vi "DeepU Front Panel.vi"() -> ()   [LabVIEW 2019, in "Results.lvlib" / "DeepU Results.lvclass"]
uses:
  DeepU Results.lvclass
  DeepU Results.lvclass/DeepU Results.ctl
  Test Stands/DeepU/DeepU Test Stand.lvclass
panel:
  out "AC":waveform(dbl)(graph) caption="Acceleration"
  out "Velocity":dbl(knob) caption="Velocity RMS, mm/s" scale=0.0..8.0
  in  "Vel":bool
  in  "AC":bool
  in  "Stable Cond":bool
  out "Inlet Pressure 2":dbl(knob) caption="Bed Pressure, kPa (g)" scale=0.0..2.0
  out "PD23 3m":dbl caption="PD 03m" format="%10.0f"
  out "PD23 1m":dbl caption="PD 01m" format="%10.0f"
  out "PD23 2m":dbl caption="PD 02m" format="%10.0f"
  out "PDX 3m":dbl format="%#10.0f"
  out "dp J 3m":dbl format="%10.0f"
  out "PDX 2m":dbl format="%#10.0f"
  out "dp J 2m":dbl format="%10.0f"
  out "PDX 1m":dbl format="%#10.0f"
  out "dp J1m":dbl format="%10.0f"
  out "TC Unit 2":string
  in  "Std Dev":bool
  out "Numeric":dbl=1.0
  in  "x std_dev":dbl=3.0 min=2.0 max=3.0 step=1.0 format="%#.0f"
  out "PDX 3 std":dbl format="%#10.0f"
  out "PDX 2 std":dbl format="%#10.0f"
  out "PDX 1 std":dbl format="%#10.0f"
  out "PDX 0 std":dbl format="%#10.0f"
  out "PD23 4 std":dbl caption="PD 4 std" format="%10.0f"
  out "PD23 1 std":dbl caption="PD 1 std" format="%10.0f"
  out "PD23 2 std":dbl caption="PD 2 std" format="%10.0f"
  out "PD23 3 std":dbl caption="PD 3 std" format="%10.0f"
  out "PD23 0 std":dbl caption="PD 0 std" format="%10.0f"
  out "J 3 std":dbl format="%10.0f"
  out "J 1 std":dbl format="%10.0f"
  out "J 2 std":dbl format="%10.0f"
  out "Fan Temp":dbl format="%#.1f"
  out "Fan Temperature":dbl(slide) scale=0.0..200.0
  out "Inv Temp":u16 caption="Inv Temp, C"
  out "Fan rpm":u16
  out "Fan I":dbl caption="Fan I, A" format="%.1f"
  out "Fan Const":bool=TRUE
  out "In range?":bool
  out "Inlet Pressure":dbl(knob) caption="Bed Pressure, kPa (g)" scale=0.0..20.0
  out "TC Unit":string
  out "paa 2":dbl caption="p bed" format="%10.0f"
  out "paa 0":dbl caption="pb" format="%10.0f"
  out "dp J 3":dbl format="%10.0f"
  out "dp J 1":dbl format="%10.0f"
  out "dp J 2":dbl format="%10.0f"
  out "PDX 2":dbl format="%#10.0f"
  out "PDX 0":dbl caption="PDX in" format="%#10.0f"
  out "PDX 1":dbl format="%#10.0f"
  out "PDX 3":dbl format="%#10.0f"
  out "Gas Humidity":dbl caption="%RH" format="%#.1f"
  out "T2":dbl format="%#5.1f"
  out "T1":dbl format="%#5.1f"
  out "Adjusted":bool
  in  "Gas Flow SP":sgl caption="Gas Flow" min=0 max=372 step=1
  in  "auto Flow":bool
  in  "Fan Out Ctrl":dbl caption="Fan Output (2 - 200 Hz)" min=0.0 max=200.0 step=1.0 format="%6.2f"
  in  "Gas Speed SP":sgl caption="Gas Speed" min=0 max=300 step=1
  out "Fan Output":dbl(slide) scale=0.0..100.0
  in  "auto":bool
  out "Gas Flow":sgl caption="Gas Flow, l/s" format="%.1f"
  out "Gas Speed":sgl caption="Gas speed" format="%10.2f"
  out "PD23 3":dbl caption="PD 03" format="%10.0f"
  out "PD23 1":dbl caption="PD 01" format="%10.0f"
  out "PD23 0":dbl caption="PD in" format="%10.0f"
  out "PD23 2":dbl caption="PD 02" format="%10.0f"
  out "PD23 4":dbl caption="PD out" format="%10.0f"
  # "Pressure in Pa"
  # "mean"
  # "dp/m"
  # "Automatic"
  # "Manual"
  # "mean"
  # "std_dev"
  # "dp/m"
  # "%"
  # "C"
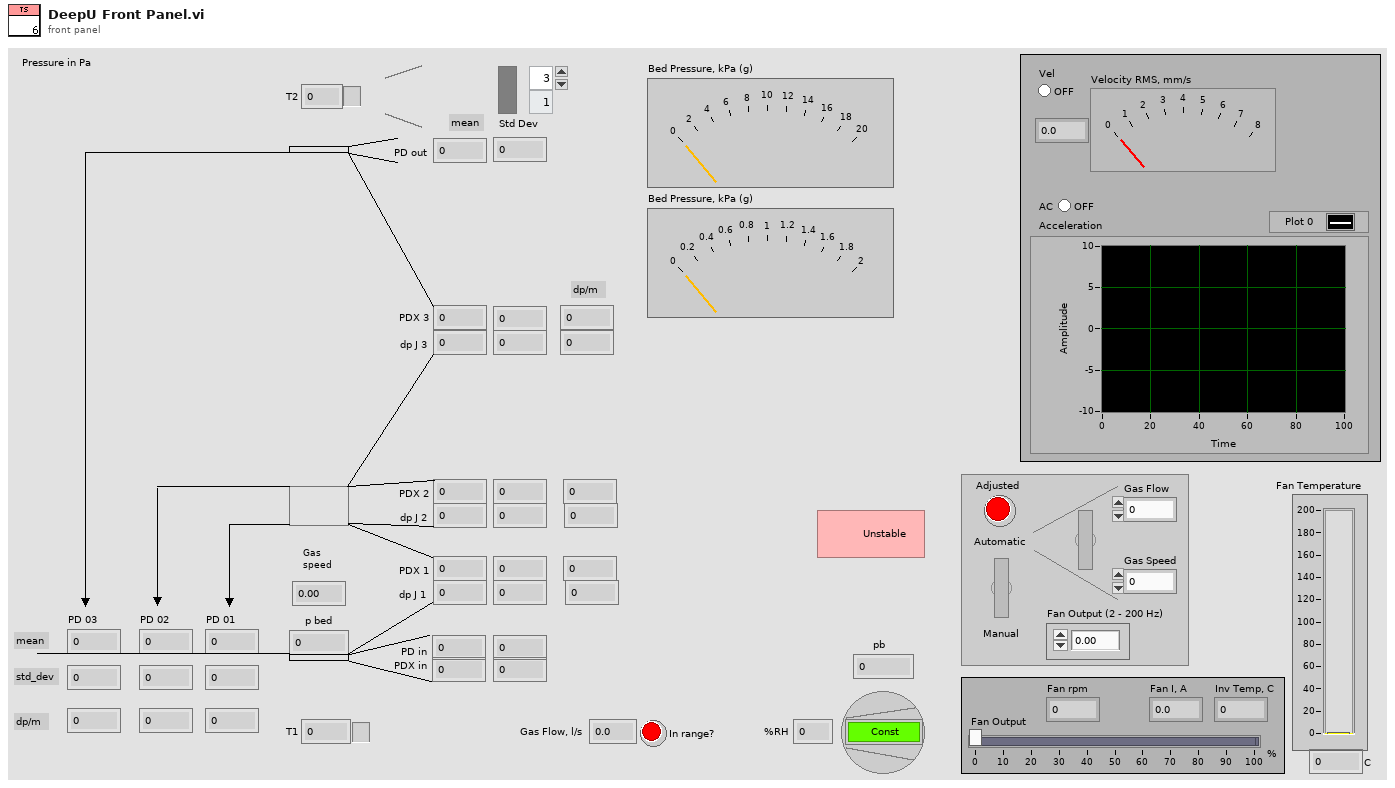
[diagram p1: front panel]
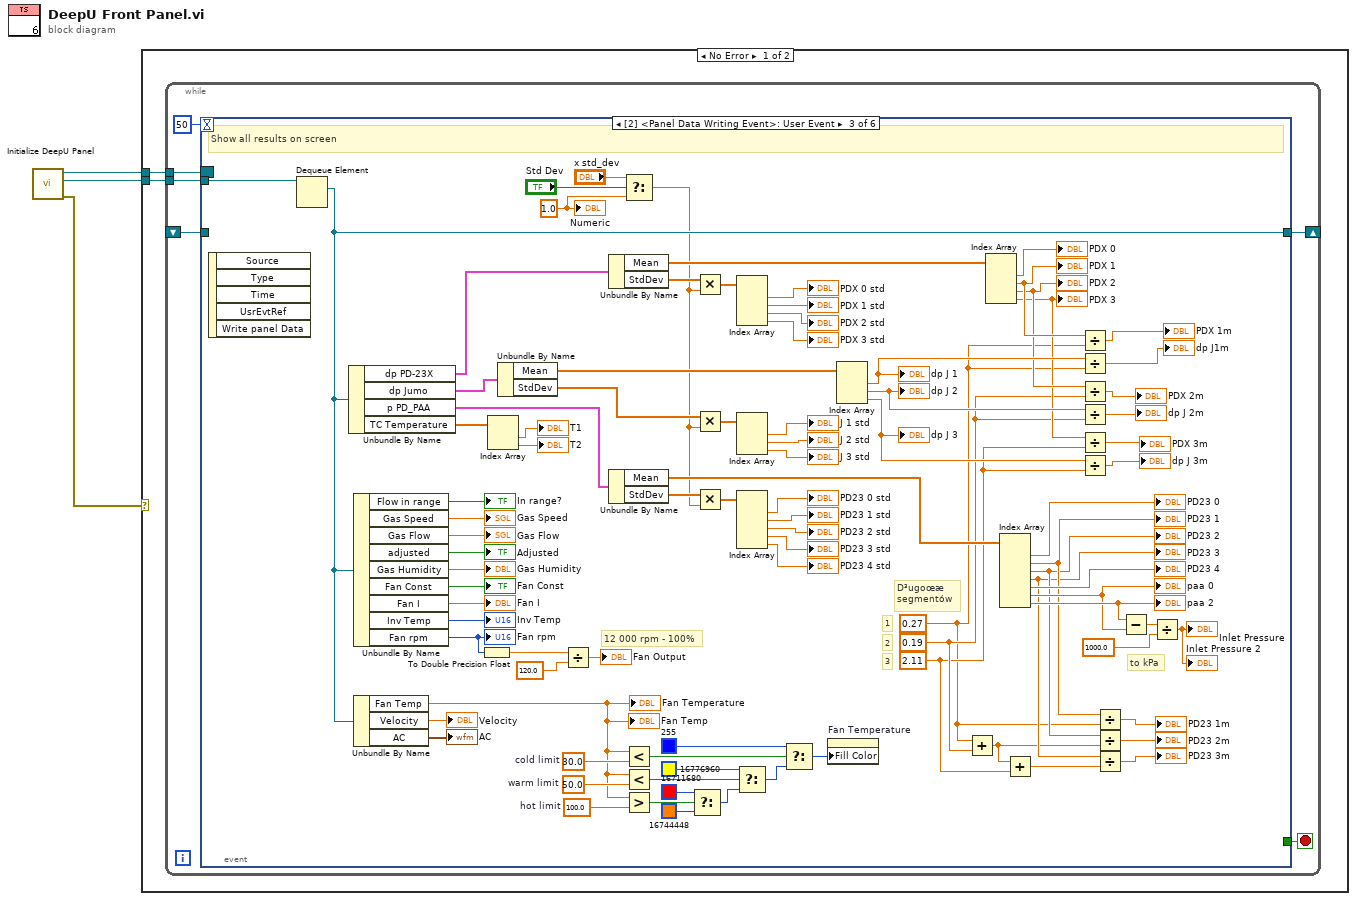
[diagram p0: block diagram]
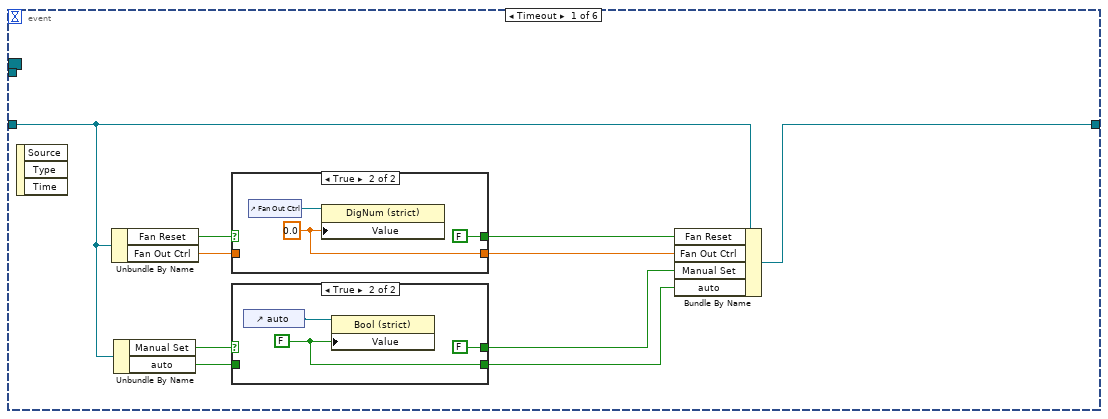
[diagram p2: hidden frame]
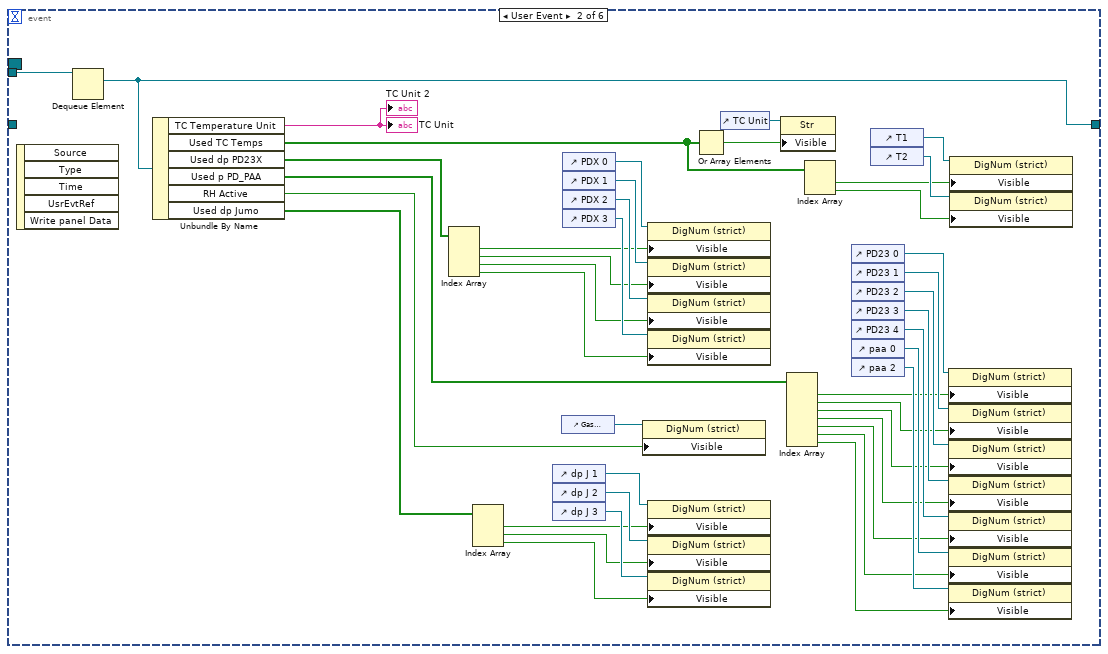
[diagram p5: hidden frame]
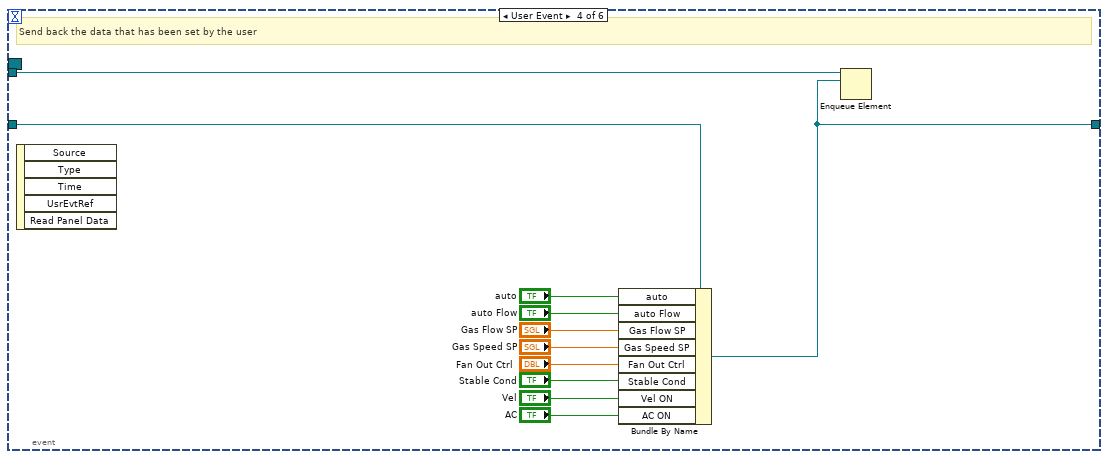
[diagram p6: hidden frame]
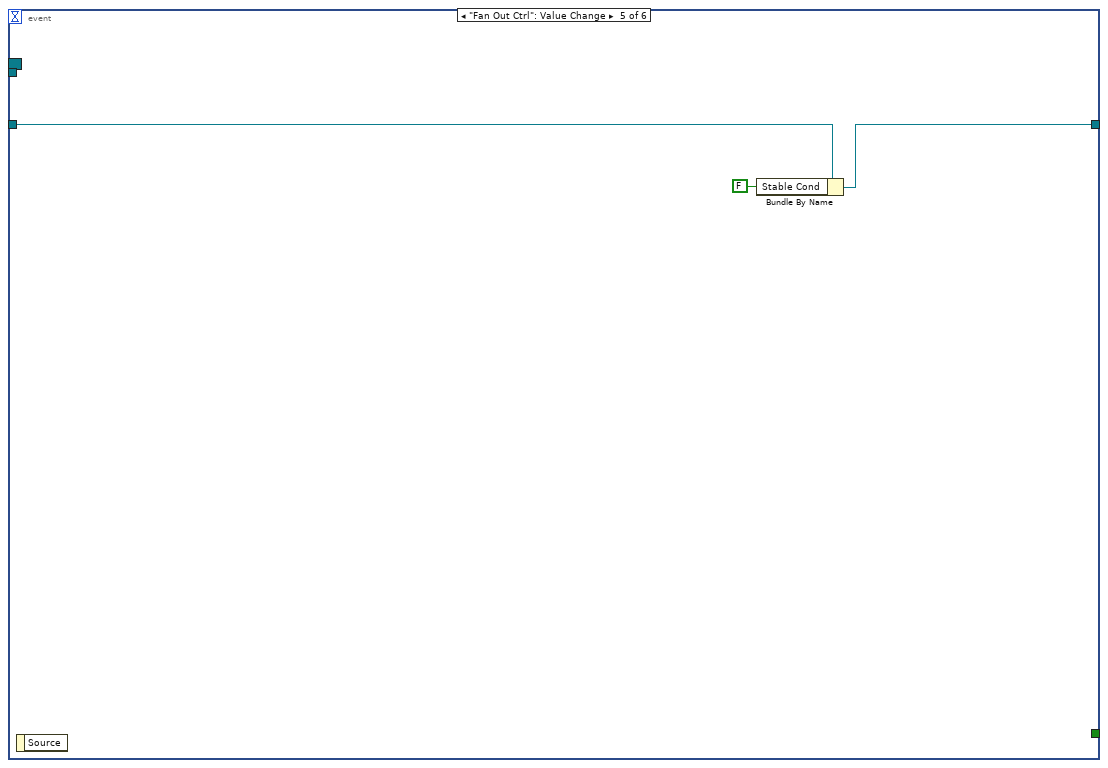
[diagram p7: hidden frame]
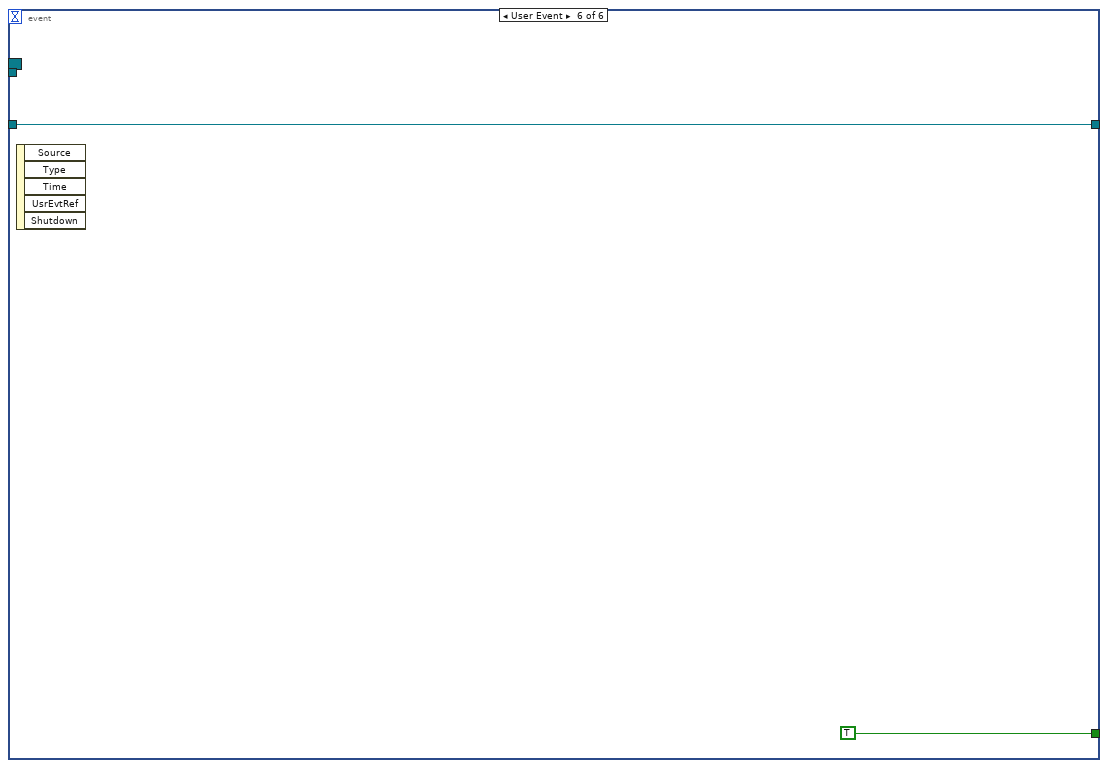
[diagram p8: hidden frame]
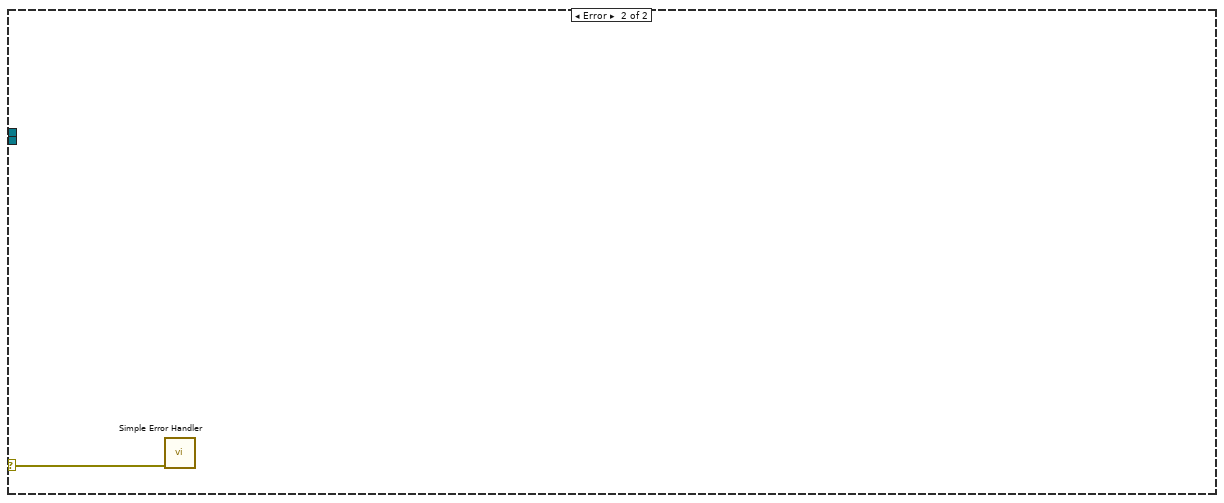
[diagram p9: hidden frame]
diagram:
  n1 = call "Initialize DeepU Panel.vi"() -> ("error out"=w3:errorcluster, "DeepU Results queue out"=w1:refnum<queue>, "Event Registration Refnum"=w2:refnum<event-registration>)  [unwired: 9 in]
  n2 = case shown="No Error" w3 {
    selector: w3 -> [_ w183]
    tunnel: w2 -> [w5 _]
    tunnel: w1 -> [w4 _]
    frame No Error {
      n3 = while {
        tunnel: w5 -> [w10]
        tunnel: w4 -> [w9]
        shift-right: [w7] -> _
        shift-left: _ -> [w6]
        stop <- w11 stop-if-true
        n4 = event shown="[2] <Panel Data Writing Event>: User Event" {
          selector: w10 -> [_ _ _ _ _ _]
          dyn-events: _ -> [_ _ _ _ _ _]
          timeout: 50 -> [_ _ _ _ _ _]
          tunnel: [_ _ _ _ _ TRUE] -> w11
          tunnel: w9 -> [_ w74 w166 w177 _ _]
          tunnel: [w21 w73 w148 w175 w179 w181] -> w7
          tunnel: w6 -> [w16 _ _ w176 w180 w181]
          event Timeout {
            n5 = event-data() -> ()  [unwired: 1 in, 3 out]
            n6 = Unbundle By Name(w16) -> ("Fan Reset"=w20:bool, "Fan Out Ctrl"=w19:dbl)
            n7 = Unbundle By Name(w16) -> ("Manual Set"=w15:bool, "auto"=w14:bool)
            n8 = case shown="True" w20 {
              selector: w20 -> [w27 _]
              tunnel: w19 -> [w28 _]
              tunnel: [w28 w29] -> w17
              tunnel: [w27 FALSE] -> w18
              frame False {
              }
              frame True {
                w29 = 0.0 ("t")
                n9 = control-ref of="Fan Out Ctrl"() -> (w31:refnum<vi>)
                n10 = property class="DigNum (strict)"(reference=w31, "Value"=w29) -> ()  [unwired: 1 in, 2 out]
              }
            }
            n11 = case shown="True" w15 {
              selector: w15 -> [w22 _]
              tunnel: w14 -> [w23 _]
              tunnel: [w23 w24] -> w12
              tunnel: [w22 FALSE] -> w13
              frame False {
              }
              frame True {
                w24 = FALSE
                n12 = control-ref of="auto"() -> (w25:refnum<vi>)
                n13 = property class="Bool (strict)"(reference=w25, "Value"=w24) -> ()  [unwired: 1 in, 2 out]
              }
            }
            n14 = Bundle By Name(cluster=w16, "Fan Reset"=w18, "Fan Out Ctrl"=w17, "Manual Set"=w13, "auto"=w12) -> (w21:refnum<class "DeepU Results.lvclass">)
          }
          event User Event {
            n15 = event-data() -> ()  [unwired: 1 in, 5 out]
            n16 = Dequeue Element(queue=w74) -> (element=w73:refnum<class "DeepU Results.lvclass">)  [unwired: 2 in, 3 out]
            n17 = Unbundle By Name(w73) -> ("TC Temperature Unit"=→"TC Unit" →"TC Unit 2":string, "Used TC Temps"=w69:bool[], "Used dp PD23X"=w64:bool[], "Used p PD_PAA"=w52:bool[], "RH Active"=w41:bool, "Used dp Jumo"=w37:bool[])
            n18 = Index Array(array=w64) -> (element #1=w63:bool, element #2=w62:bool, element #3=w61:bool, element #4=w60:bool)  [unwired: 4 in]
            n19 = Index Array(array=w37) -> (element #1=w36:bool, element #2=w35:bool, element #3=w34:bool)  [unwired: 3 in]
            n20 = control-ref of="dp J 1"() -> (w40:refnum<vi>)
            n21 = control-ref of="dp J 2"() -> (w39:refnum<vi>)
            n22 = control-ref of="dp J 3"() -> (w38:refnum<vi>)
            n23 = control-ref of="Gas Humidity"() -> (w44:refnum<vi>)
            n24 = control-ref of="PDX 0"() -> (w68:refnum<vi>)
            n25 = control-ref of="PDX 1"() -> (w67:refnum<vi>)
            n26 = control-ref of="PDX 2"() -> (w66:refnum<vi>)
            n27 = control-ref of="PDX 3"() -> (w65:refnum<vi>)
            n28 = property class="DigNum (strict)"(reference=w44, "Visible"=w41) -> ()  [unwired: 1 in, 2 out]
            n29 = property class="DigNum (strict)"(reference=w68, "Visible"=w63) -> ()  [unwired: 1 in, 2 out]
            n30 = property class="DigNum (strict)"(reference=w67, "Visible"=w62) -> ()  [unwired: 1 in, 2 out]
            n31 = property class="DigNum (strict)"(reference=w66, "Visible"=w61) -> ()  [unwired: 1 in, 2 out]
            n32 = property class="DigNum (strict)"(reference=w65, "Visible"=w60) -> ()  [unwired: 1 in, 2 out]
            n33 = property class="DigNum (strict)"(reference=w40, "Visible"=w36) -> ()  [unwired: 1 in, 2 out]
            n34 = property class="DigNum (strict)"(reference=w39, "Visible"=w35) -> ()  [unwired: 1 in, 2 out]
            n35 = property class="DigNum (strict)"(reference=w38, "Visible"=w34) -> ()  [unwired: 1 in, 2 out]
            n36 = Or Array Elements(Boolean array=w69) -> (logical OR=w43:bool)
            n37 = control-ref of="TC Unit"() -> (w72:refnum<vi>)
            n38 = property class="Str"(reference=w72, "Visible"=w43) -> ()  [unwired: 1 in, 2 out]
            n39 = Index Array(array=w52) -> (element #1=w51:bool, element #2=w45:bool, element #3=w46:bool, element #4=w47:bool, element #5=w48:bool, element #6=w49:bool, element #7=w50:bool)  [unwired: 7 in]
            n40 = Index Array(array=w69) -> (element #1=w42:bool, element #2=w33:bool)  [unwired: 2 in]
            n41 = control-ref of="PD23 0"() -> (w59:refnum<vi>)
            n42 = control-ref of="PD23 1"() -> (w58:refnum<vi>)
            n43 = control-ref of="PD23 2"() -> (w57:refnum<vi>)
            n44 = control-ref of="PD23 3"() -> (w56:refnum<vi>)
            n45 = control-ref of="PD23 4"() -> (w55:refnum<vi>)
            n46 = control-ref of="paa 0"() -> (w54:refnum<vi>)
            n47 = control-ref of="paa 2"() -> (w53:refnum<vi>)
            n48 = control-ref of="T1"() -> (w70:refnum<vi>)
            n49 = control-ref of="T2"() -> (w71:refnum<vi>)
            n50 = property class="DigNum (strict)"(reference=w59, "Visible"=w51) -> ()  [unwired: 1 in, 2 out]
            n51 = property class="DigNum (strict)"(reference=w58, "Visible"=w45) -> ()  [unwired: 1 in, 2 out]
            n52 = property class="DigNum (strict)"(reference=w57, "Visible"=w46) -> ()  [unwired: 1 in, 2 out]
            n53 = property class="DigNum (strict)"(reference=w56, "Visible"=w47) -> ()  [unwired: 1 in, 2 out]
            n54 = property class="DigNum (strict)"(reference=w55, "Visible"=w48) -> ()  [unwired: 1 in, 2 out]
            n55 = property class="DigNum (strict)"(reference=w54, "Visible"=w49) -> ()  [unwired: 1 in, 2 out]
            n56 = property class="DigNum (strict)"(reference=w53, "Visible"=w50) -> ()  [unwired: 1 in, 2 out]
            n57 = property class="DigNum (strict)"(reference=w70, "Visible"=w42) -> ()  [unwired: 1 in, 2 out]
            n58 = property class="DigNum (strict)"(reference=w71, "Visible"=w33) -> ()  [unwired: 1 in, 2 out]
          }
          event User Event {
            w80 = 2.11 ("y")
            w82 = 0.19 ("y")
            w78 = 0.27 ("y")
            w103 = 1.0 ("Numeric")
            w146 = 100.0  # hot limit
            w150 = 50.0  # warm limit
            w152 = 30.0  # cold limit
            # "3"
            # "2"
            # "1"
            # "D³ugoœæ\nsegmentów"
            # "to kPa"
            # "12 000 rpm - 100%"
            # "Show all results on screen"
            n59 = event-data() -> ()  [unwired: 1 in, 5 out]
            n60 = Dequeue Element(queue=w166) -> (element=w148:refnum<class "DeepU Results.lvclass">)  [unwired: 2 in, 3 out]
            n61 = Unbundle By Name(w148) -> ("dp PD-23X"=w162:cluster{"Mean":dbl[], "StdDev":dbl[]}, "dp Jumo"=w135:cluster{"Mean":dbl[], "StdDev":dbl[]}, "p PD_PAA"=w112:cluster{"Mean":dbl[], "StdDev":dbl[]}, "TC Temperature"=w111:dbl[])
            n62 = Unbundle By Name(w148) -> ("Flow in range"=→"In range?":bool, "Gas Speed"=→"Gas Speed":sgl, "Gas Flow"=→"Gas Flow":sgl, "adjusted"=→"Adjusted":bool, "Gas Humidity"=→"Gas Humidity":dbl, "Fan Const"=→"Fan Const":bool, "Fan I"=→"Fan I":dbl, "Inv Temp"=→"Inv Temp":u16, "Fan rpm"=w154:u16)
            "Fan rpm" <- w154
            n63 = Unbundle By Name(w148) -> ("Fan Temp"=w138:dbl, "Velocity"=→"Velocity":dbl, "AC"=→"AC":waveform(dbl))
            "Fan Temperature" <- w138
            "Fan Temp" <- w138
            n64 = To Double Precision Float(number=w154) -> (double precision float=w153:dbl)
            n65 = Index Array(array=w111) -> (element #1=→"T1":dbl, element #2=→"T2":dbl)  [unwired: 2 in]
            n66 = Unbundle By Name(w135) -> ("Mean"=w134:dbl[], "StdDev"=w108:dbl[])
            n67 = Divide(x=w153, y=120.0) -> (x/y=→"Fan Output":dbl)
            n68 = Unbundle By Name(w162) -> ("Mean"=w125:dbl[], "StdDev"=w106:dbl[])
            n69 = Unbundle By Name(w112) -> ("Mean"=w124:dbl[], "StdDev"=w110:dbl[])
            n70 = Select(t="x std_dev", s="Std Dev", f=w103) -> (s? t:f=w101:dbl)
            n71 = Less?(x=w138, y=w152) -> (x < y?=w151:bool)
            n72 = Less?(x=w138, y=w150) -> (x < y?=w149:bool)
            n73 = Greater?(x=w138, y=w146) -> (0:w147:bool)
            n74 = Select(t=u32 16711680 ("Fill Color"), s=w147, f=u32 16744448 ("Fill Color")) -> (s? t:f=w140:u32)
            n75 = Multiply(x=w106, y=w101) -> (x*y=w105:dbl[])
            n76 = Multiply(x=w108, y=w101) -> (x*y=w107:dbl[])
            n77 = Multiply(x=w110, y=w101) -> (x*y=w109:dbl[])
            n78 = Index Array(array=w105) -> (element #1=→"PDX 0 std":dbl, element #2=→"PDX 1 std":dbl, element #3=→"PDX 2 std":dbl, element #4=→"PDX 3 std":dbl)  [unwired: 4 in]
            n79 = Index Array(array=w107) -> (element #1=→"J 1 std":dbl, element #2=→"J 2 std":dbl, element #3=→"J 3 std":dbl)  [unwired: 3 in]
            n80 = Index Array(array=w109) -> (element #1=→"PD23 0 std":dbl, element #2=→"PD23 1 std":dbl, element #3=→"PD23 2 std":dbl, element #4=→"PD23 3 std":dbl, element #5=→"PD23 4 std":dbl)  [unwired: 5 in]
            n81 = Select(t=u32 16776960 ("Fill Color"), s=w149, f=w140) -> (s? t:f=w145:u32)
            n82 = Select(t=u32 255 ("Fill Color"), s=w151, f=w145) -> (s? t:f=w139:u32)
            n83 = property on="Fan Temperature" class="Slide (strict)"("Fill Color"=w139) -> ()  [unwired: 2 in, 2 out]
            n84 = Index Array(array=w134) -> (element #1=w98:dbl, element #2=w94:dbl, element #3=w91:dbl)  [unwired: 3 in]
            "dp J 3" <- w91
            "dp J 1" <- w98
            "dp J 2" <- w94
            n85 = Add(x=w78, y=w82) -> (x+y=w81:dbl)
            n86 = Index Array(array=w125) -> (element #1=→"PDX 0":dbl, element #2=w100:dbl, element #3=w95:dbl, element #4=w92:dbl)  [unwired: 4 in]
            "PDX 2" <- w95
            "PDX 1" <- w100
            "PDX 3" <- w92
            n87 = Index Array(array=w124) -> (element #1=→"PD23 0":dbl, element #2=w85:dbl, element #3=w84:dbl, element #4=w83:dbl, element #5=→"PD23 4":dbl, element #6=w122:dbl, element #7=w123:dbl)  [unwired: 7 in]
            "PD23 2" <- w84
            "PD23 1" <- w85
            "PD23 3" <- w83
            "paa 0" <- w122
            "paa 2" <- w123
            n88 = Add(x=w81, y=w80) -> (x+y=w79:dbl)
            n89 = Divide(x=w100, y=w78) -> (x/y=→"PDX 1m":dbl)
            n90 = Divide(x=w98, y=w78) -> (x/y=→"dp J1m":dbl)
            n91 = Divide(x=w95, y=w82) -> (x/y=→"PDX 2m":dbl)
            n92 = Divide(x=w94, y=w82) -> (x/y=→"dp J 2m":dbl)
            n93 = Divide(x=w92, y=w80) -> (x/y=→"PDX 3m":dbl)
            n94 = Divide(x=w91, y=w80) -> (x/y=→"dp J 3m":dbl)
            n95 = Divide(x=w85, y=w78) -> (x/y=→"PD23 1m":dbl)
            n96 = Divide(x=w84, y=w81) -> (x/y=→"PD23 2m":dbl)
            n97 = Divide(x=w83, y=w79) -> (x/y=→"PD23 3m":dbl)
            n98 = Subtract(x=w123, y=w122) -> (x-y=w137:dbl)
            n99 = Divide(x=w137, y=1000.0) -> (x/y=→"Inlet Pressure" →"Inlet Pressure 2":dbl)
            "Numeric" <- w103
          }
          event User Event {
            # "Send back the data that has been set by the user"
            n100 = event-data() -> ()  [unwired: 1 in, 5 out]
            n101 = Bundle By Name(cluster=w176, "auto"="auto", "auto Flow"="auto Flow", "Gas Flow SP"="Gas Flow SP", "Gas Speed SP"="Gas Speed SP", "Fan Out Ctrl"="Fan Out Ctrl", "Stable Cond"="Stable Cond", "Vel ON"="Vel", "AC ON"="AC") -> (w175:refnum<class "DeepU Results.lvclass">)
            n102 = Enqueue Element(queue=w177, element=w175) -> ()  [unwired: 2 in, 3 out]
          }
          event "Fan Out Ctrl": Value Change {
            n103 = event-data() -> ()  [unwired: 1 in, 1 out]
            n104 = Bundle By Name(cluster=w180, "Stable Cond"=FALSE) -> (w179:refnum<class "DeepU Results.lvclass">)
          }
          event User Event {
            n105 = event-data() -> ()  [unwired: 1 in, 5 out]
          }
        }
      }
    }
    frame Error {
      n106 = call <vilib>:"Simple Error Handler.vi"("error in (no error)"=w183) -> ()  [unwired: 4 in, 5 out]
    }
  }
